vi "RFH-average-libreVNA.vi"(7 "Source Folder":path, 8 "error in (no error)":errorcluster) -> (0 "error out":errorcluster, 2 "Common Format":T1)   [LabVIEW 2020, in "RFH-Reflection_File_Handler.lvlib"]
doc: "Reads every LibreVNA file in a folder and averages them into one Common Format cluster."
uses:
  RFH-Reflection_File_Handler.lvlib
  RFH-common_data_format.ctl
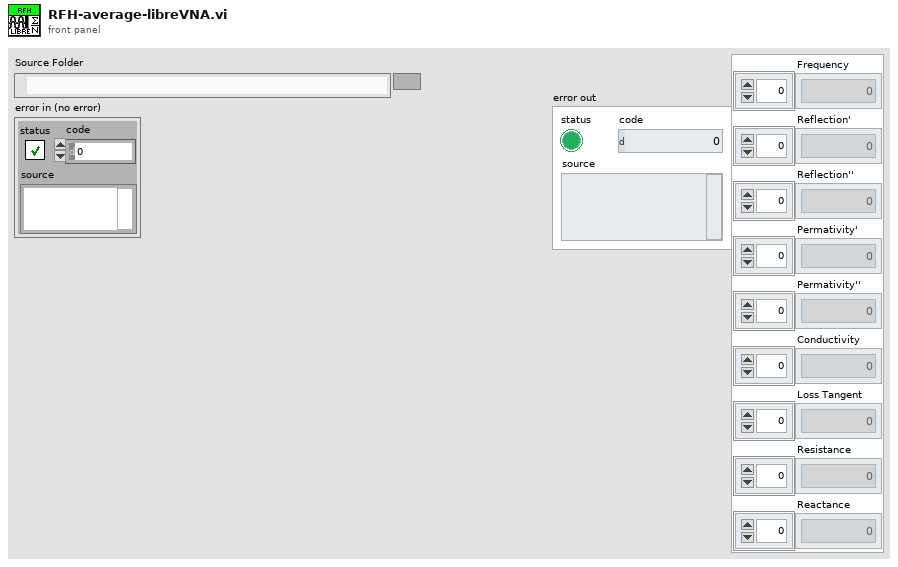
[diagram p1: front panel]
types:
  T1 = typedef "RFH-Reflection_File_Handler.lvlib/RFH-common_data_format.ctl" = cluster{"Frequency":dbl[], "Reflection'":dbl[], "Reflection''":dbl[], "Permativity'":dbl[], "Permativity''":dbl[], "Conductivity":dbl[], "Loss Tangent":dbl[], "Resistance":dbl[], "Reactance":dbl[]}
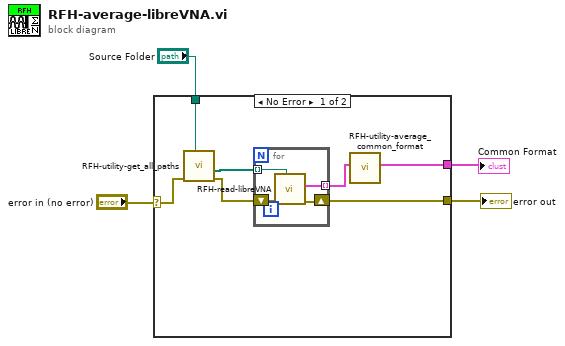
[diagram p0: block diagram]
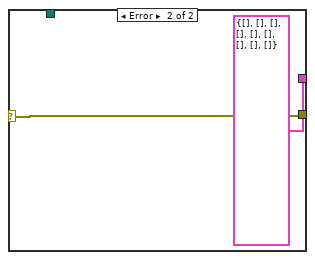
[diagram p2: hidden frame]
diagram:
  n1 = case shown="No Error" "error in (no error)" {
    selector: "error in (no error)" -> [w7 w17]
    tunnel: "Source Folder" -> [w8 _]
    tunnel: [w6 w17] -> w2
    tunnel: [w5 T1 {"Frequency"=[], "Reflection'"=[], "Reflection''"=[], "Permativity'"=[], "Permativity''"=[], "Conductivity"=[], "Loss Tangent"=[], "Resistance"=[], "Reactance"=[]} ("Common Format")] -> w1
    frame No Error {
      n2 = call "RFH-utility-get_all_paths.vi"("Folder Path"=w8, "error in (no error)"=w7) -> ("error out"=w9:errorcluster, "All Files in Dir"=w11:path[])  [unwired: 6 in, 2 out]
      n3 = for {
        tunnel: w11 -> [w13] mode=indexing
        tunnel: [w12] -> w10 mode=indexing
        shift-right: [w14] -> w6
        shift-left: w9 -> [w15]
        n4 = call "RFH-read-libreVNA.vi"("file path (dialog if empty)"=w13, "error in"=w15) -> ("error out"=w14:errorcluster, "Common Format"=w12:T1)  [unwired: 8 in]
      }
      n5 = call "RFH-utility-average_common_format.vi"("common array in"=w10) -> ("Common Format"=w5:T1)  [unwired: 10 in]
    }
    frame Error {
    }
  }
  "error out" <- w2
  "Common Format" <- w1
